vi "RemoteVI Is Button Down.vi"(0 "posts":cluster{"msg":u32, "wParam":u64, "lParam":i64}[](array[cluster])) -> (4 "button down?":bool)   [LabVIEW 2020, in "RemoteVI.lvlib"]
doc: "TRUE when the first message in posts is a mouse button-down or double click (WM_LBUTTONDOWN, WM_LBUTTONDBLCLK, WM_RBUTTONDOWN, WM_RBUTTONDBLCLK, WM_MBUTTONDOWN, WM_MBUTTONDBLCLK). Pure."
uses:
  RemoteVI.lvlib
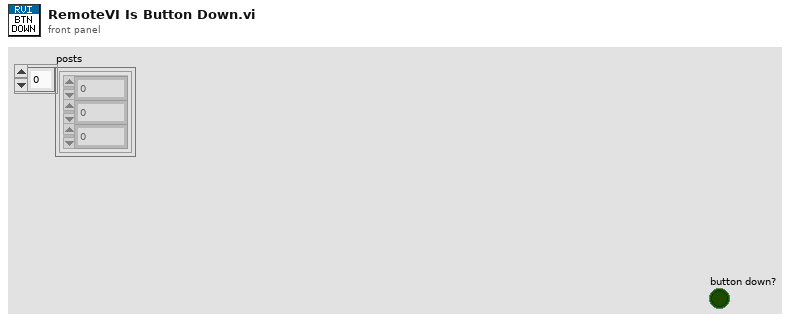
[diagram p1: front panel]
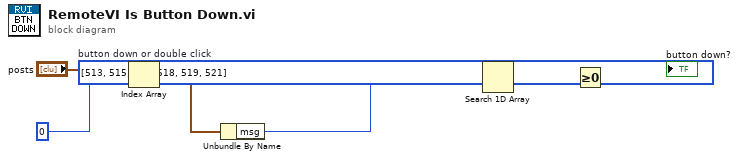
[diagram p0: block diagram]
diagram:
  w5 = u32[] [513, 515, 516, 518, 519, 521]  # button down or double click
  n1 = Index Array(array="posts", index=0) -> (element=w3:cluster{"msg":u32, "wParam":u64, "lParam":i64})
  n2 = Unbundle By Name(w3) -> ("msg"=w4:u32)
  n3 = Search 1D Array(1D array=w5, element=w4) -> (index of element=w6:i32)  [unwired: 1 in]
  n4 = Greater Or Equal To 0?(x=w6) -> (x >= 0?=→"button down?":bool)
